vi "SetPanel.vi"(8 "error in (no error)":errorcluster, 11 "ChannelManagerUI in":refnum<class "ChannelManagerUI.lvclass">) -> (0 "error out":errorcluster, 3 "ChannelManagerUI out":refnum<class "ChannelManagerUI.lvclass">)   [LabVIEW 2021, in "Channel.lvlib" / "ChannelManagerUI.lvlib" / "ChannelManagerUI.lvclass"]
uses:
  ChannelManagerUI.lvclass
  Channel_class/Channel.lvclass
  ChannelManagerUI.lvclass/ChannelManagerUI.ctl
  Configuration_class/Configuration.lvclass
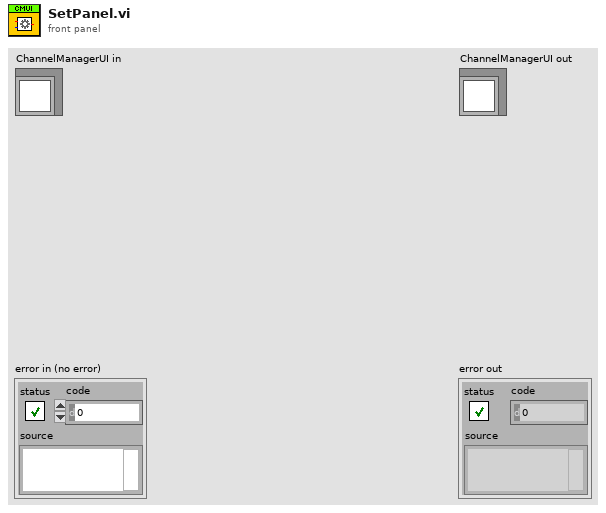
[diagram p1: front panel]
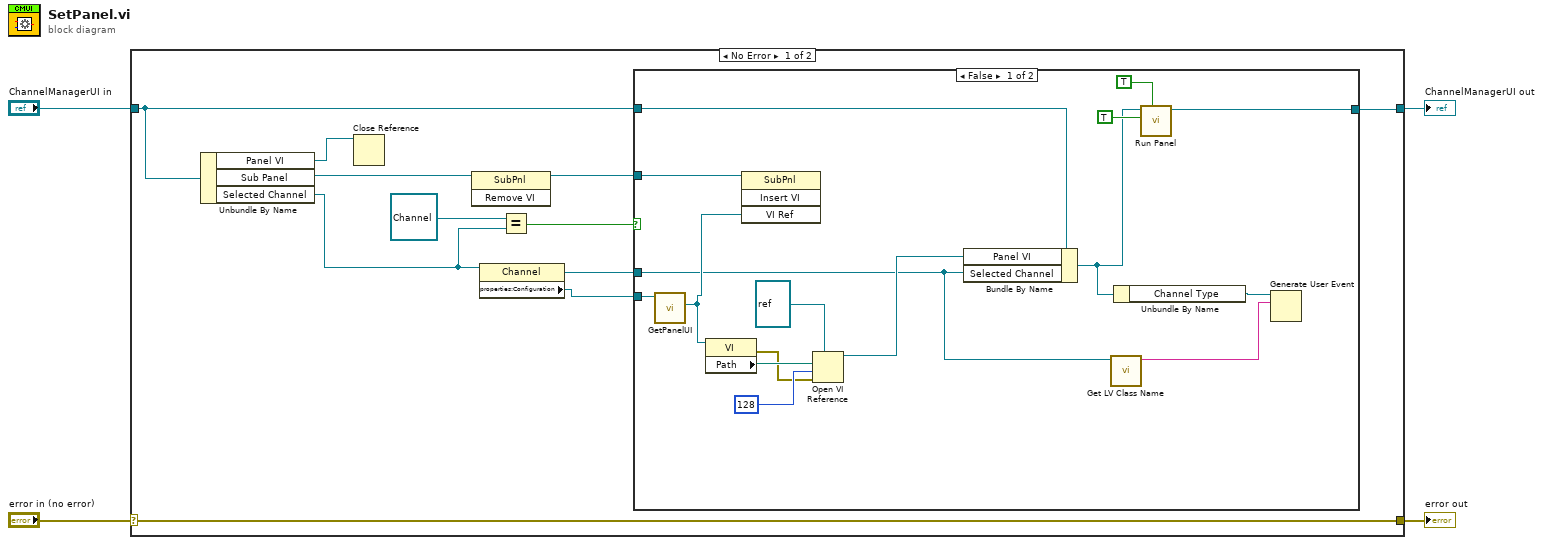
[diagram p0: block diagram]
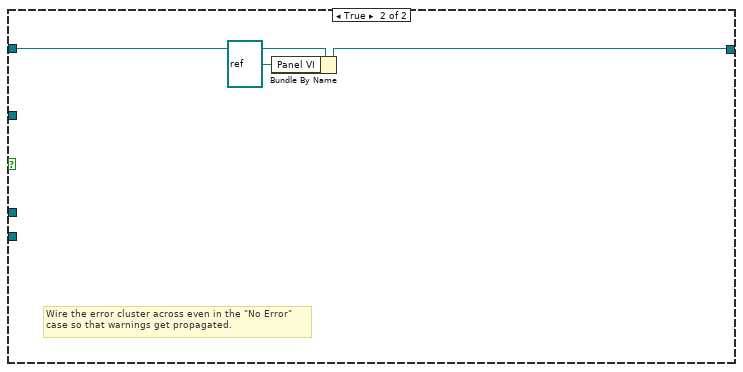
[diagram p2: hidden frame]
diagram:
  n1 = case shown="No Error" "error in (no error)" {
    selector: "error in (no error)" -> [w15 w36]
    tunnel: [w15 w36] -> w3
    tunnel: [w7 w35] -> w1
    tunnel: "ChannelManagerUI in" -> [w8 w35]
    frame No Error {
      n2 = Unbundle By Name(w8) -> ("Panel VI"=w6:refnum<vi>, "Sub Panel"=w14:refnum<vi>, "Selected Channel"=w12:refnum<class "Channel.lvclass">)
      n3 = Close Reference(reference=w6) -> ()  [unwired: 1 in, 1 out]
      n4 = invoke class="SubPnl" method="Remove VI"(reference=w14) -> (reference out=w10:refnum<vi>)  [unwired: 2 in, 2 out]
      n5 = property class="Channel"(reference=w12) -> (reference out=w9:refnum<class "Channel.lvclass">, "properties:Configuration"=w5:refnum<class "Configuration.lvclass">)  [unwired: 1 in, 1 out]
      n6 = Equal?(x=refnum<class "Channel.lvclass"> refnum ("Selected Channel"), y=w12) -> (x = y?=w11:bool)
      n7 = case shown="False" w11 {
        tunnel: w10 -> [w31 _]
        tunnel: w9 -> [w19 _]
        tunnel: w8 -> [w30 w34]
        tunnel: [w24 w33] -> w7
        tunnel: w5 -> [w21 _]
        frame False {
          n8 = call-dynamic "GetPanelUI.vi"("object in"=w21) -> ("VI Refnum"=w20:refnum<vi>)  [unwired: 8 in, 2 out]
          n9 = property class="VI"(reference=w20) -> (error out=w26:errorcluster, "Path"=w29:path)  [unwired: 1 in, 1 out]
          n10 = invoke class="SubPnl" method="Insert VI"(reference=w31, "VI Ref"=w20) -> ()  [unwired: 2 in, 4 out]
          n11 = Open VI Reference(type specifier VI Refnum (for type only)=refnum<vi> refnum, vi path=w29, options=128, error in (no error)=w26) -> (vi reference=w25:refnum<vi>)  [unwired: 2 in, 1 out]
          n12 = Bundle By Name(cluster=w30, "Panel VI"=w25, "Selected Channel"=w19) -> (w18:refnum<class "ChannelManagerUI.lvclass">)
          n13 = call <vilib>:"Get LV Class Name.vi"("object"=w19) -> ("class name"=w16:string)  [unwired: 9 in, 1 out]
          n14 = Unbundle By Name(w18) -> ("Channel Type"=w17:refnum<user-event>)
          n15 = call "Run Panel.vi"("Set(F)"=TRUE, "First Time(F)"=TRUE, "ChannelManagerUI in"=w18) -> ("ChannelManagerUI out"=w24:refnum<class "ChannelManagerUI.lvclass">)  [unwired: 5 in, 3 out]
          n16 = Generate User Event(user event=w17, event data cluster=w16) -> ()  [unwired: 2 in, 2 out]
        }
        frame True {
          # "Wire the error cluster across even in the \"No Error\"\ncase so that warnings get propagated."
          n17 = Bundle By Name(cluster=w34, "Panel VI"=refnum<vi> refnum) -> (w33:refnum<class "ChannelManagerUI.lvclass">)
        }
      }
    }
    frame Error {
    }
  }
  "error out" <- w3
  "ChannelManagerUI out" <- w1
